vi "[ce] LM Fit - ABX.vi"(5 "Standard Deviation ^2":dbl[](array[numeric]), 6 "error in":errorcluster, 7 "data for given coefficients":dbl[](array[numeric]), 8 "Y":dbl[](array[numeric]), 9 "coefficient values":dbl[](array[numeric])) -> (0 "error out":errorcluster, 2 "Beta":dbl[](array[numeric]), 3 "Alpha":dbl[][](array[numeric]))   [LabVIEW 2021]
doc: "::: CalcExpress Toolkit :::\nCopyright (c) 2000-2026 Konstantin Shifershteyn. All rights reserved."
uses:
  <vilib>/Analysis/baseanly.llb/Real Outer Product.vi
  <vilib>/Analysis/NI_AALBase.lvlib
  cersrc/celveng32.dll
panel:
  in  "Use CIN (T)":bool=TRUE
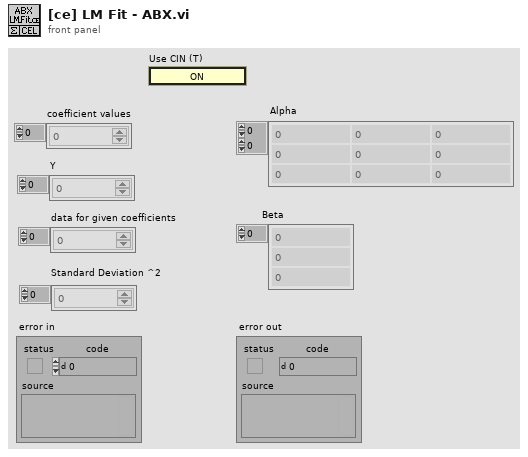
[diagram p1: front panel]
types:
  T1 = typedef "NI_Matrix.lvlib/RealMatrix.ctl" = dbl[][]
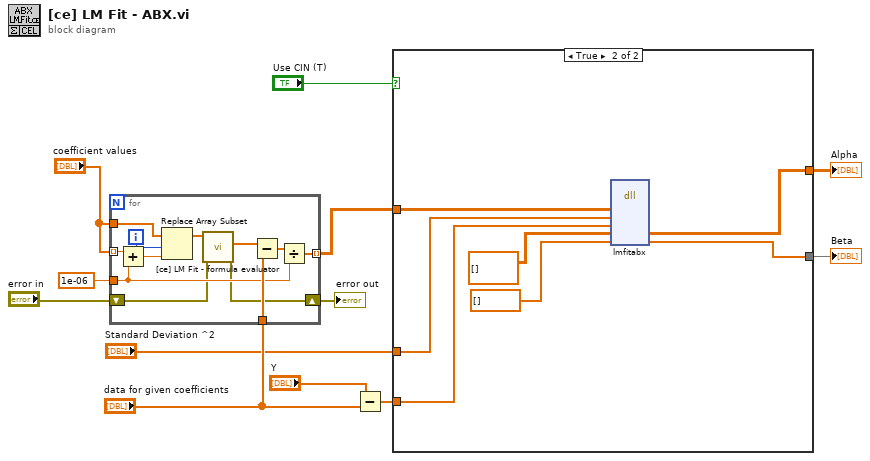
[diagram p0: block diagram]
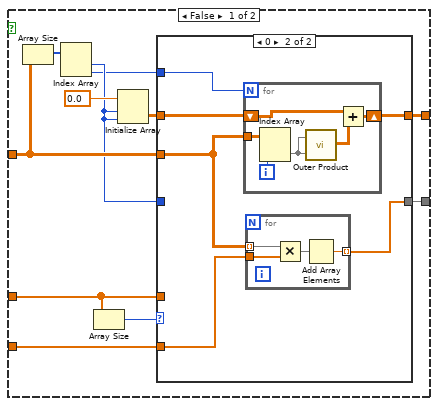
[diagram p2: hidden frame]
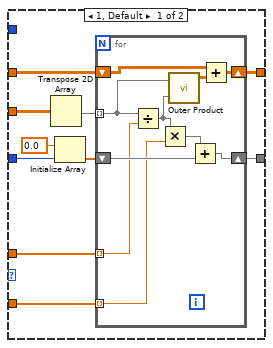
[diagram p3: hidden frame]
diagram:
  n1 = for {
    tunnel: "coefficient values" -> [w22]
    tunnel: "coefficient values" -> [w21] mode=indexing
    tunnel: 1e-06 -> [w16]
    tunnel: "data for given coefficients" -> [w19]
    tunnel: [w17] -> w2 mode=indexing
    shift-right: [w15] -> w10
    shift-left: "error in" -> [w14]
    i -> [w23]
    n2 = Add(x=w21, y=w16) -> (x+y=w24:dbl)
    n3 = Replace Array Subset(array=w22, new element=w24, index=w23) -> (w13:dbl[])
    n4 = call "[ce] LM Fit - formula evaluator.vi"("error in"=w14, "coef values"=w13) -> ("error out"=w15:errorcluster, "calc result"=w20:dbl[])  [unwired: 7 in, 1 out]
    n5 = Subtract(x=w20, y=w19) -> (x-y=w18:dbl[])
    n6 = Divide(x=w18, y=w16) -> (x/y=w17:dbl[])
  }
  "error out" <- w10
  n7 = Subtract(x="Y", y="data for given coefficients") -> (x-y=w3:dbl[])
  n8 = case shown="True" "Use CIN (T)" {
    tunnel: [w33 w76] -> w6
    tunnel: [w31 w75] -> w5
    tunnel: "Standard Deviation ^2" -> [w30 w73]
    tunnel: w3 -> [w29 w72]
    tunnel: w2 -> [w27 w74]
    frame False {
      n9 = Array Size(array=w27) -> (size(s)=w28:i32[])
      n10 = Index Array(array=w28) -> (element #1=w26:i32, element #2=w25:i32)  [unwired: 2 in]
      n11 = Array Size(array=w30) -> (size(s)=w34:i32)
      n12 = Initialize Array(0.0, w26, w26) -> (w32:dbl[][])
      n13 = case shown="0" w34 {
        tunnel: w32 -> [w45 w58]
        tunnel: [w44 w57] -> w31
        tunnel: [w43 w60] -> w33
        tunnel: w29 -> [w42 w61]
        tunnel: w30 -> [w41 _]
        tunnel: w27 -> [w36 w59]
        tunnel: w26 -> [w38 _]
        tunnel: w25 -> [_ w56]
        frame 1, Default {
          n14 = Transpose 2D Array(2D array=w36) -> (transposed array=w37:dbl[][])
          n15 = Initialize Array(0.0, w38) -> (w39:dbl[])
          n16 = for {
            shift-right: [w54] -> w43
            shift-left: w39 -> [w55]
            shift-right: [w49] -> w44
            shift-left: w45 -> [w50]
            tunnel: w37 -> [w47] mode=indexing
            tunnel: w42 -> [w53] mode=indexing
            tunnel: w41 -> [w51] mode=indexing
            n17 = Divide(x=w47, y=w51) -> (x/y=w46:dbl[])
            n18 = Multiply(x=w46, y=w53) -> (x*y=w52:dbl[])
            n19 = call-poly <vilib>:"Outer Product.vi"("Y Vector"=w46, "X Vector"=w47) -> ("Outer Product"=w48:T1)  [unwired: 1 out]
            n20 = Add(x=w52, y=w55) -> (x+y=w54:dbl[])
            n21 = Add(x=w50, y=w48) -> (x+y=w49:T1)
          }
        }
        frame 0 {
          n22 = for {
            N: w56 -> [_]
            shift-right: [w64] -> w57
            shift-left: w58 -> [w65]
            tunnel: w59 -> [w63]
            i -> [w62]
            n23 = Index Array(array=w63, index (col)=w62) -> (element=w67:dbl[])  [unwired: 1 in]
            n24 = call-poly <vilib>:"Outer Product.vi"("Y Vector"=w67, "X Vector"=w67) -> ("Outer Product"=w66:T1)  [unwired: 1 out]
            n25 = Add(x=w65, y=w66) -> (x+y=w64:T1)
          }
          n26 = for {
            tunnel: w59 -> [w71] mode=indexing
            tunnel: w61 -> [w70]
            tunnel: [w68] -> w60 mode=indexing
            n27 = Multiply(x=w71, y=w70) -> (x*y=w69:dbl[])
            n28 = Add Array Elements(numeric array=w69) -> (sum=w68:dbl)
          }
        }
      }
    }
    frame True {
      n29 = dll-call lib="C:/LV Projects/CalcExpress 40 LV2021/vi.lib/addons/CalcExpress/cersrc/celveng*.dll" fn="lmfitabx"("in_VAR"=w74, "in_STD"=w73, "in_DIF"=w72, "out_Alpha"=dbl[][] [] ("input"), "out_Beta"=dbl[] [] ("input")) -> ("out_Alpha"=w75:dbl[][], "out_Beta"=w76:dbl[])  [unwired: 7 in, 2 out]
    }
  }
  "Alpha" <- w5
  "Beta" <- w6
